vi "Write INI Table.vi"(6 "Keys":string[](array[string]), 7 "Table Name":string, 8 "error in (no error)":errorcluster, 9 "Values":string[][](array[string]), 10 "Section Names":string[](array[string]), 11 "File Path":path) -> (0 "error out":errorcluster)   [LabVIEW 2024]
doc: "Writes a whole schema-version-2 INI file - a FULL REWRITE, so rows that are no longer in the table disappear from the file. The file starts with [_Meta] holding Schema Version = 2 and Table = the given table name, followed by one section per row: the section name is the row key from Section Names and each of the Keys becomes one line with the value from Values (one row of Values per section, one column per key).\n\nA key name prefixed with # is written as a number and one prefixed with ? as a boolean (TRUE/FALSE), both without quotes and without the prefix; every other value is written as a quoted, escaped string. That matches what LabVIEW's configuration file VIs write.\n\nGenerated by: Claude"
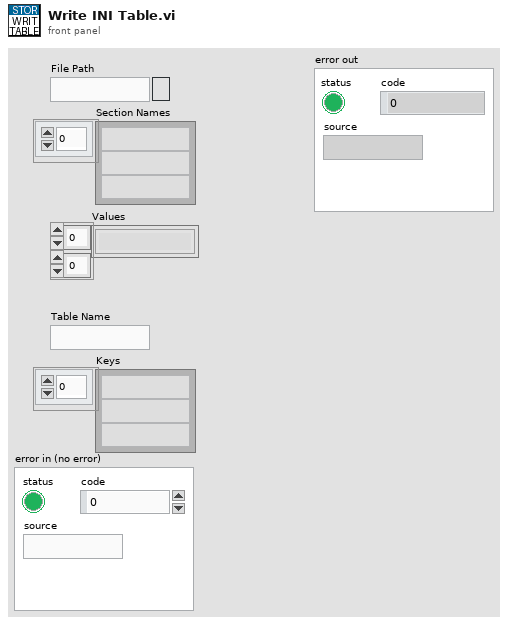
[diagram p1: front panel]
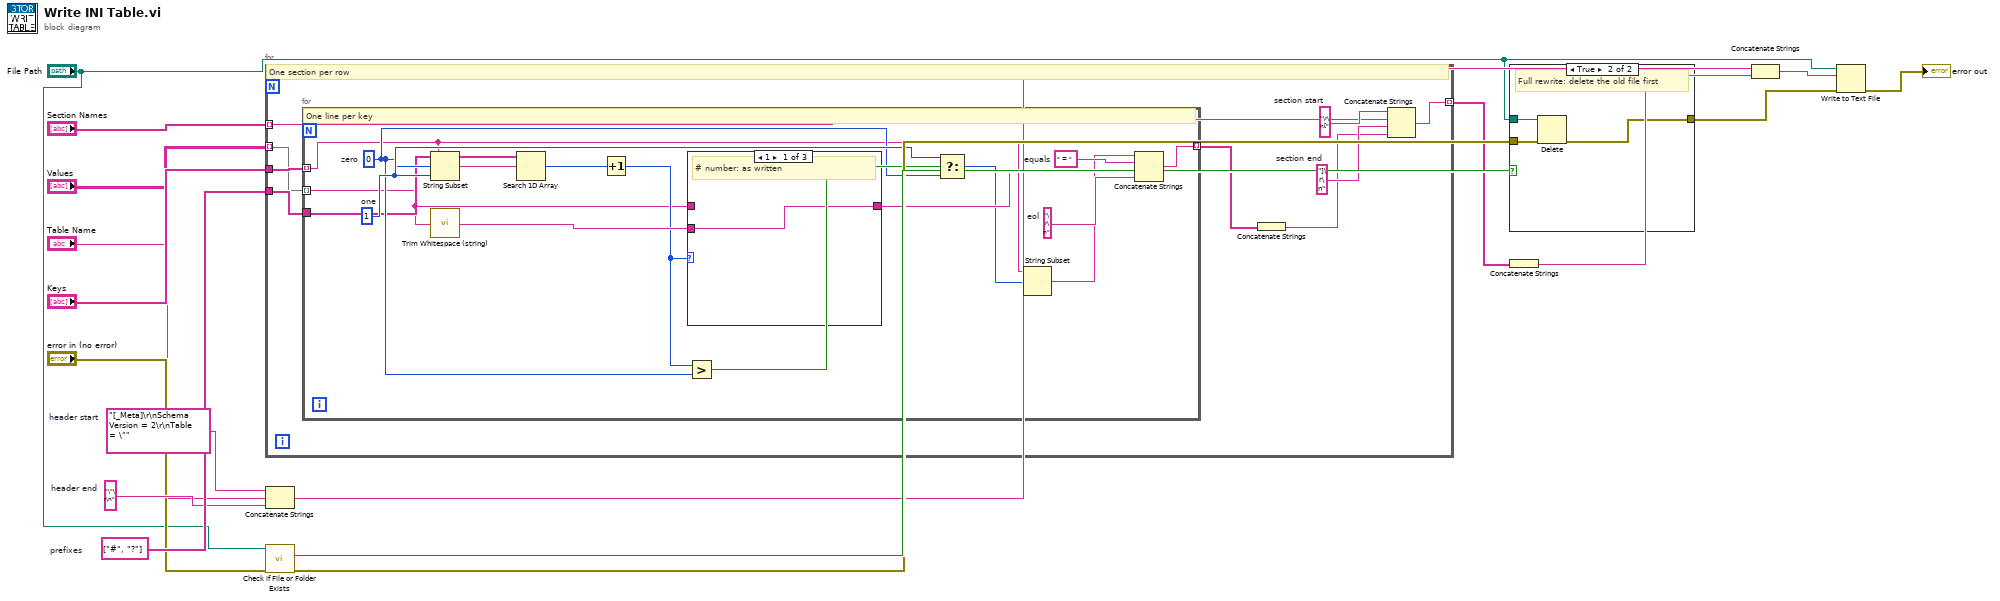
[diagram p0: block diagram]
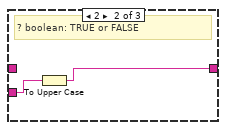
[diagram p3: hidden frame]
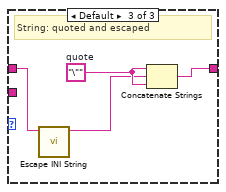
[diagram p4: hidden frame]
diagram:
  w10 = string[] ["#", "?"]  # prefixes
  w8 = "\"\r\n"  # header end
  w7 = "[_Meta]\r\nSchema Version = 2\r\nTable = \""  # header start
  n1 = for {
    tunnel: "Section Names" -> [w18] mode=indexing
    tunnel: "Values" -> [w19] mode=indexing
    tunnel: "Keys" -> [w20]
    tunnel: w10 -> [w21]
    tunnel: [w26] -> w11 mode=indexing
    w25 = "]\r\n"  # section end
    w24 = "\r\n["  # section start
    # "One section per row"
    n2 = for {
      tunnel: w20 -> [w27] mode=indexing
      tunnel: w19 -> [w28] mode=indexing
      tunnel: w21 -> [w29]
      tunnel: [w42] -> w22 mode=indexing
      w41 = "\r\n"  # eol
      w40 = " = "  # equals
      w31 = 1  # one
      w30 = 0  # zero
      # "One line per key"
      n3 = String Subset(string=w27, offset (0)=w30, length (rest)=w31) -> (substring=w32:string)
      n4 = call <vilib>:"Trim Whitespace (string).vi"("string"=w28) -> ("trimmed string"=w38:string)  [unwired: 1 in]
      n5 = Search 1D Array(1D array=w29, element=w32) -> (index of element=w33:i32)  [unwired: 1 in]
      n6 = Increment(x=w33) -> (x+1=w34:i32)
      n7 = case shown="1" w34 {
        tunnel: w28 -> [_ _ w46]
        tunnel: w38 -> [w43 w44 _]
        tunnel: [w43 w45 w49] -> w39
        frame 1 {
          # "# number: as written"
        }
        frame 2 {
          # "? boolean: TRUE or FALSE"
          n8 = To Upper Case(1:w44) -> (0:w45:string)
        }
        frame Default {
          w48 = "\""  # quote
          # "String: quoted and escaped"
          n9 = call "Escape INI String.vi"("Text"=w46) -> ("Escaped"=w47:string)  [unwired: 9 in, 1 out]
          n10 = Concatenate Strings(w48, w47, w48) -> (w49:string)
        }
      }
      n11 = Greater?(x=w34, y=w30) -> (0:w35:bool)
      n12 = Select(t=w31, s=w35, f=w30) -> (s? t:f=w36:i32)
      n13 = String Subset(string=w27, offset (0)=w36) -> (substring=w37:string)  [unwired: 1 in]
      n14 = Concatenate Strings(w37, w40, w39, w41) -> (w42:string)
    }
    n15 = Concatenate Strings(w22) -> (w23:string)
    n16 = Concatenate Strings(w24, w18, w25, w23) -> (w26:string)
  }
  n17 = Concatenate Strings(w7, "Table Name", w8) -> (w9:string)
  n18 = call <vilib>:"Check if File or Folder Exists.vi"("error in (no error)"="error in (no error)", "path"="File Path") -> ("error out"=w14:errorcluster, "file or folder exists?"=w15:bool)  [unwired: 7 in, 1 out]
  n19 = case shown="True" w15 {
    tunnel: "File Path" -> [_ w51]
    tunnel: w14 -> [w50 w52]
    tunnel: [w50 w53] -> w16
    frame False {
    }
    frame True {
      # "Full rewrite: delete the old file first"
      n20 = Delete(path (use dialog)=w51, error in=w52) -> (error out=w53:errorcluster)  [unwired: 3 in, 2 out]
    }
  }
  n21 = Concatenate Strings(w11) -> (w12:string)
  n22 = Concatenate Strings(w9, w12) -> (w13:string)
  n23 = Write to Text File(file (use dialog)="File Path", text=w13, error in=w16) -> (error out=→"error out":errorcluster)  [unwired: 1 in, 2 out]
